vi "VIH ProjFile - XML - Property Element - Create.vi"(8 "error in":errorcluster, 10 "Property Name":string, 11 "XML Parent Item":refnum<k20>) -> (0 "error out":errorcluster, 2 "New Child":refnum<k20>, 3 "dup XML Parent Item":refnum<k20>)   [LabVIEW 2014]
doc: "::: VI Helpeks :::\nCopyright (c) 2000-2026 Konstantin Shifershteyn. All rights reserved."
uses:
  <resource>/objmgr/DOMUserDefRef.rc
panel:
  # "VI Helpeks\nCopyright (c) 2012-2026 Konstantin Shifershteyn"
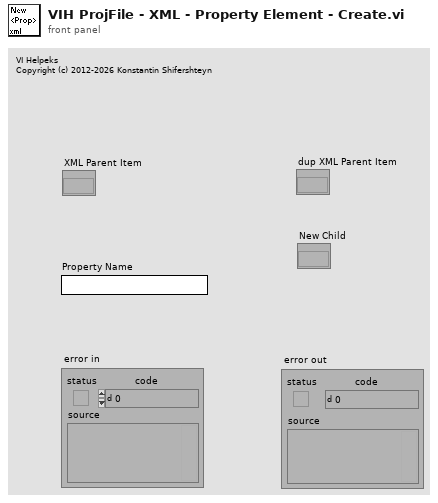
[diagram p1: front panel]
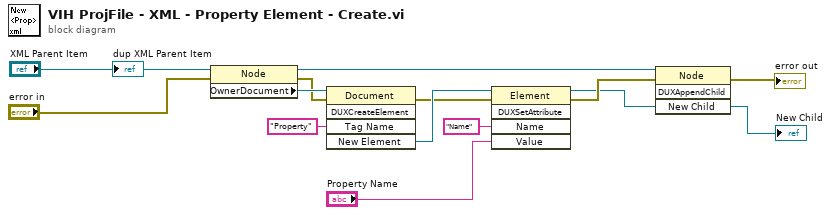
[diagram p0: block diagram]
diagram:
  n1 = property class="Node"(reference="XML Parent Item", error in="error in") -> (reference out=w10:refnum<k20>, error out=w7:errorcluster, "OwnerDocument"=w11:refnum<k20>)
  n2 = invoke class="Document" method="DUXCreateElement"(reference=w11, error in=w7, "Tag Name"="Property") -> (error out=w6:errorcluster, "New Element"=w8:refnum<k20>)  [unwired: 2 in, 3 out]
  n3 = invoke class="Element" method="DUXSetAttribute"(reference=w8, error in=w6, "Name"="Name", "Value"="Property Name") -> (reference out=w2:refnum<k20>, error out=w4:errorcluster)  [unwired: 1 in, 3 out]
  "New Child" <- w2
  n4 = invoke class="Node" method="DUXAppendChild"(reference=w10, error in=w4, "New Child"=w2) -> (error out=→"error out":errorcluster)  [unwired: 1 in, 3 out]
  "dup XML Parent Item" <- "XML Parent Item"
